vi "[ce] Open VIT dynamic instance.vi"(6 "error in":errorcluster, 8 "VI instance name":string, 9 "VI template path":path) -> (0 "error out":errorcluster, 3 "vi refnum":refnum<vi>, 4 "new window?":bool)   [LabVIEW 2021]
doc: "### DEPRECATED ###\n\n::: CalcExpress Toolkit :::\nCopyright (c) 2000-2026 Konstantin Shifershteyn. All rights reserved."
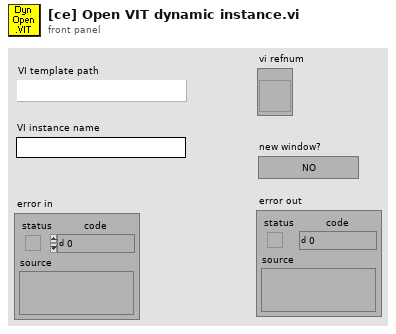
[diagram p1: front panel]
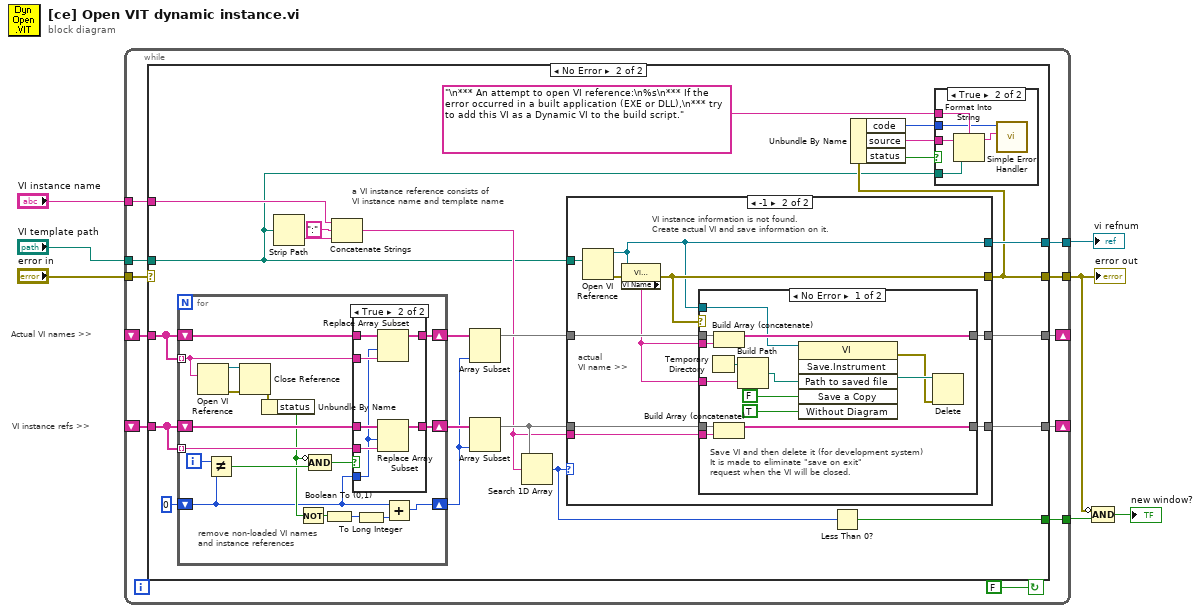
[diagram p0: block diagram]
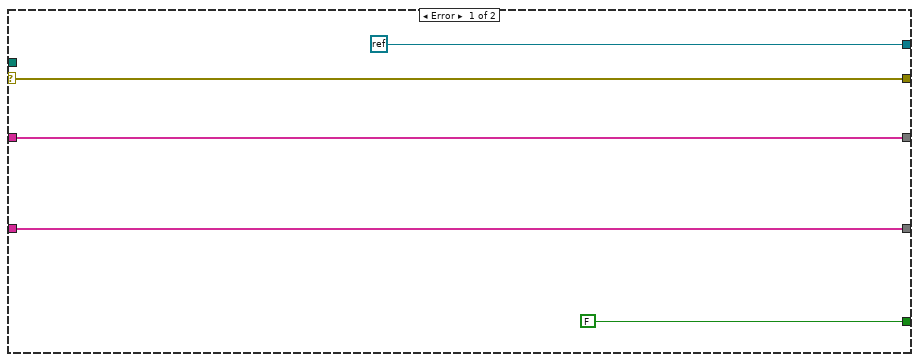
[diagram p2: hidden frame]
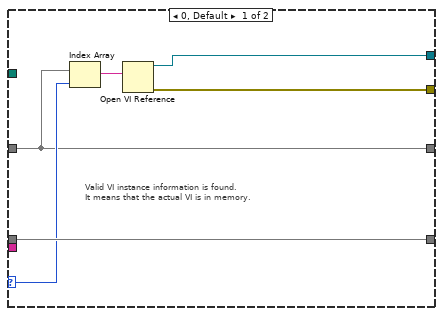
[diagram p4: hidden frame]
diagram:
  # "VI instance refs >>"
  # "Actual VI names >>"
  n1 = while {
    tunnel: [w12] -> w4
    tunnel: [w13] -> w6
    tunnel: [w14] -> w3
    tunnel: "error in" -> [w10]
    shift-left: _ -> [w18]
    shift-right: [w15] -> _
    shift-left: _ -> [w17]
    shift-right: [w16] -> _
    tunnel: "VI instance name" -> [w9]
    tunnel: "VI template path" -> [w8]
    stop <- FALSE continue-if-true
    n2 = case shown="No Error" w10 {
      selector: w10 -> [w19 _]
      tunnel: w18 -> [w22 w34]
      tunnel: w17 -> [w23 w33]
      tunnel: [w23 w40] -> w16
      tunnel: [w22 w38] -> w15
      tunnel: [w19 w26] -> w14
      tunnel: [refnum<k0> refnum w35] -> w13
      tunnel: [FALSE w32] -> w12
      tunnel: w9 -> [_ w25]
      tunnel: w8 -> [_ w24]
      frame Error {
      }
      frame No Error {
        # "a VI instance reference consists of\nVI instance name and template name"
        n3 = for {
          shift-right: [w97] -> w44
          shift-left: w34 -> [w96]
          shift-right: [w84] -> w43
          shift-left: 0 -> [w83]
          shift-right: [w95] -> w45
          shift-left: w33 -> [w91]
          tunnel: w34 -> [w90] mode=indexing
          tunnel: w33 -> [w89] mode=indexing
          i -> [w92]
          # "remove non-loaded VI names\nand instance references"
          n4 = Open VI Reference(vi path=w89) -> (vi reference=w100:refnum<vi>, error out=w99:errorcluster)  [unwired: 5 in]
          n5 = Not Equal?(x=w92, y=w83) -> (x != y?=w94:bool)
          n6 = Close Reference(reference=w100, error in (no error)=w99) -> (error out=w98:errorcluster)
          n7 = Unbundle By Name(w98) -> ("status"=w88:bool)
          n8 = Not(x=w88) -> (.not. x?=w87:bool)
          n9 = Compound Arithmetic op=AND(invert w88, w94) -> (w93:bool)
          n10 = Boolean To (0,1)(Boolean=w87) -> (0, 1=w86:i16)
          n11 = case shown="True" w93 {
            tunnel: w96 -> [w102 w109]
            tunnel: [w102 w108] -> w97
            tunnel: w90 -> [_ w107]
            tunnel: w91 -> [w101 w106]
            tunnel: [w101 w105] -> w95
            tunnel: w89 -> [_ w104]
            tunnel: w83 -> [_ w103]
            frame False {
            }
            frame True {
              n12 = Replace Array Subset(array=w106, new element=w104, index=w103) -> (w105:string[])
              n13 = Replace Array Subset(array=w109, new element=w107, index=w103) -> (w108:string[])
            }
          }
          n14 = To Long Integer(number=w86) -> (32bit integer=w85:i32)
          n15 = Add(x=w83, y=w85) -> (x+y=w84:i32)
        }
        n16 = Strip Path(path=w24) -> (name=w41:string)  [unwired: 1 out]
        n17 = Concatenate Strings(w25, ":", w41) -> (w36:string)
        n18 = Array Subset(array=w45, length=w43) -> (w39:string[])  [unwired: 1 in]
        n19 = Array Subset(array=w44, length=w43) -> (w37:string[])  [unwired: 1 in]
        n20 = Search 1D Array(1D array=w37, element=w36) -> (index of element=w31:i32)  [unwired: 1 in]
        n21 = case shown="-1" w31 {
          selector: w31 -> [w56 _]
          tunnel: w24 -> [_ w66]
          tunnel: [w55 w65] -> w40
          tunnel: w39 -> [w55 w64]
          tunnel: w37 -> [w57 w62]
          tunnel: [w57 w63] -> w38
          tunnel: w36 -> [_ w61]
          tunnel: [w53 w59] -> w26
          tunnel: [w52 w58] -> w35
          frame 0, Default {
            # "Valid VI instance information is found.\nIt means that the actual VI is in memory."
            n22 = Index Array(array=w55, index=w56) -> (element=w54:string)
            n23 = Open VI Reference(vi path=w54) -> (vi reference=w52:refnum<vi>, error out=w53:errorcluster)  [unwired: 5 in]
          }
          frame -1 {
            # "VI instance information is not found.\nCreate actual VI and save information on it."
            # "actual\nVI name >>"
            n24 = Open VI Reference(vi path=w66) -> (vi reference=w58:refnum<vi>, error out=w67:errorcluster)  [unwired: 5 in]
            n25 = property on="vi name" class="VirtualInstrument"(reference=w58, error in=w67) -> (error out=w59:errorcluster, "VI Name"=w60:string)  [unwired: 1 out]
            n26 = case shown="No Error" w59 {
              tunnel: [w80 w82] -> w65
              tunnel: w64 -> [w79 w82]
              tunnel: w60 -> [w78 _]
              tunnel: [w77 w81] -> w63
              tunnel: w62 -> [w76 w81]
              tunnel: w61 -> [w75 _]
              tunnel: w60 -> [w69 _]
              tunnel: w58 -> [w68 _]
              frame No Error {
                # "Save VI and then delete it (for development system)\nIt is made to eliminate \"save on exit\"\nrequest when the VI will be closed."
                n27 = Temporary Directory() -> (w70:path)
                n28 = Build Array (concatenate)(w79, w78) -> (w80:string[])
                n29 = Build Array (concatenate)(w76, w75) -> (w77:string[])
                n30 = Build Path(base path=w70, name or relative path=w69) -> (appended path=w74:path)
                n31 = invoke class="VI" method="Save.Instrument"(reference=w68, "Path to saved file"=w74, "Save a Copy"=FALSE, "Without Diagram"=TRUE) -> (error out=w73:errorcluster)  [unwired: 2 in, 5 out]
                n32 = Delete(path (use dialog)=w74, error in=w73) -> ()  [unwired: 3 in, 3 out]
              }
              frame Error {
              }
            }
          }
        }
        n33 = Less Than 0?(x=w31) -> (x < 0?=w32:bool)
        n34 = Unbundle By Name(w26) -> ("code"=w29:i32, "source"=w30:string, "status"=w28:bool)
        n35 = case shown="True" w28 {
          tunnel: w30 -> [_ w51]
          tunnel: w24 -> [_ w50]
          tunnel: "\n*** An attempt to open VI reference:\n%s\n*** If the error occurred in a built application (EXE or DLL),\n*** try to add this VI as a Dynamic VI to the build script." -> [_ w49]
          tunnel: w29 -> [_ w48]
          frame False {
          }
          frame True {
            n36 = Format Into String(format string=w49, initial string=w51, w50) -> (resulting string=w47:string)  [unwired: 1 in, 1 out]
            n37 = call <vilib>:"Simple Error Handler.vi"("error code (no error:0)"=w48, "error source (\" \")"=w47) -> ()  [unwired: 3 in, 5 out]
          }
        }
      }
    }
  }
  "error out" <- w3
  "vi refnum" <- w6
  n38 = Compound Arithmetic op=AND(invert w3, w4) -> (→"new window?":bool)
